vi "Node LUT.vi"(6 "Command":T2, 8 "error in":errorcluster, 9 "node ref":T1, 10 "UID":string) -> (0 "error out":errorcluster, 1 "node ref":T1, 2 "node refs":T1[](array[typedef]), 3 "UIDs":string[](array[string]))   [LabVIEW 2015, in "Node LUT.lvlib"]
uses:
  Node LUT.lvlib
  Command.ctl
  <vilib>/NI/Configuration Framework/Node/NodeRef.ctl
  <vilib>/NI/Configuration Framework/Node/NISE_CEF_Node.lvclass
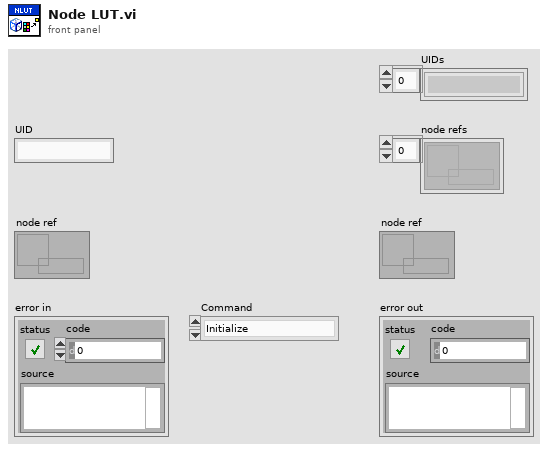
[diagram p1: front panel]
types:
  T1 = typedef "NISE_CEF_Node.lvclass/NodeRef.ctl" = refnum<data-value>
  T2 = typedef "Node LUT.lvlib/Command.ctl" = enum16{"Initialize", "Add Node", "Remove Node", "Node Ref from UID", "List Nodes"}
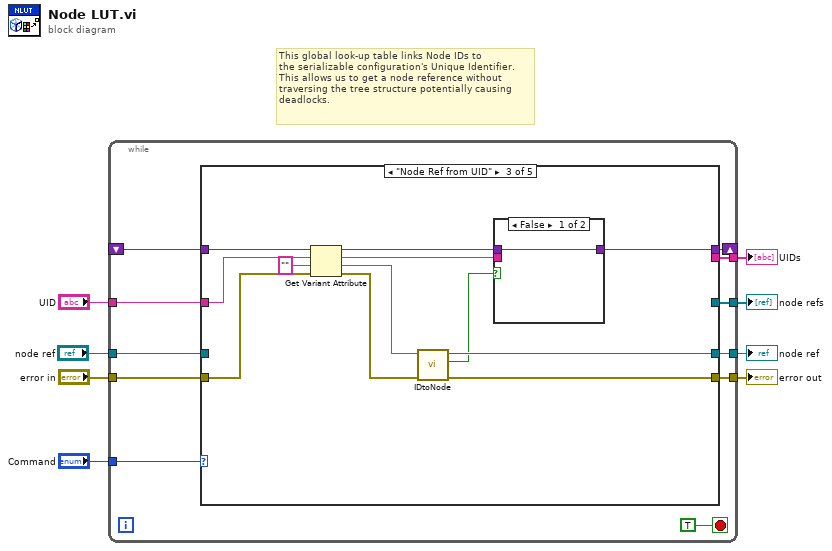
[diagram p0: block diagram]
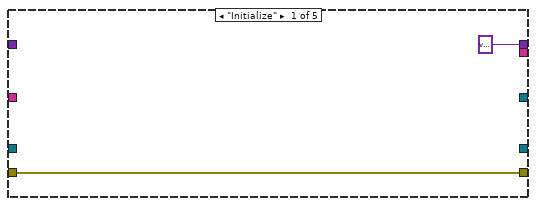
[diagram p2: hidden frame]
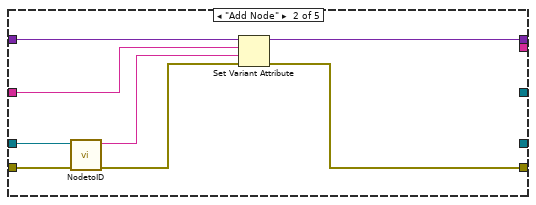
[diagram p3: hidden frame]
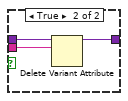
[diagram p4: hidden frame]
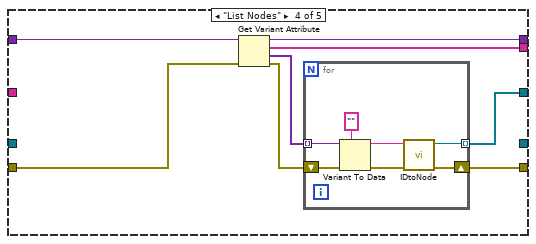
[diagram p5: hidden frame]
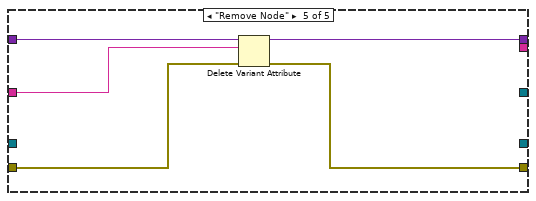
[diagram p6: hidden frame]
diagram:
  # "This global look-up table links Node IDs to\nthe serializable configuration's Unique Identifier.\nThis allows us to get a node reference without\ntraversing the tree structure potentially causing\ndeadlocks."
  n1 = while {
    tunnel: "Command" -> [w18]
    shift-right: [w17] -> _
    shift-left: _ -> [w16]
    tunnel: [w15] -> w7
    tunnel: "error in" -> [w14]
    tunnel: "UID" -> [w13]
    tunnel: "node ref" -> [w12]
    tunnel: [w11] -> w3
    tunnel: [w10] -> w2
    tunnel: [w9] -> w1
    stop <- TRUE stop-if-true
    n2 = case shown="\"Node Ref from UID\"" w18 {
      tunnel: [variant w28 w31 w51 w64] -> w17
      tunnel: w16 -> [_ w29 w40 w52 w60]
      tunnel: [w20 w27 w36 w48 w63] -> w15
      tunnel: w14 -> [w20 w25 w39 w50 w62]
      tunnel: w13 -> [_ w26 w32 _ w61]
      tunnel: w12 -> [_ w22 _ _ _]
      tunnel: [_ _ _ w46 _] -> w11
      tunnel: [_ _ _ w45 _] -> w10
      tunnel: [_ _ w34 _ _] -> w9
      frame "Initialize" {
      }
      frame "Add Node" {
        n3 = call <vilib>:"NodetoID.vi"("error in"=w25, "node ref"=w22) -> ("error out"=w24:errorcluster, "ID"=w23:string)  [unwired: 8 in]
        n4 = Set Variant Attribute(Variant=w29, name=w26, value=w23, error in=w24) -> (Variant out=w28:variant, error out=w27:errorcluster)  [unwired: 1 out]
      }
      frame "Node Ref from UID" {
        n5 = Get Variant Attribute(Variant=w40, name=w32, default value (empty Variant)="", error in=w39) -> (duplicate Variant=w33:variant, value=w35:string, error out=w37:errorcluster)  [unwired: 1 out]
        n6 = call <vilib>:"IDtoNode.vi"("error in"=w37, "ID"=w35) -> ("error out"=w36:errorcluster, "invalid Id"=w30:bool, "node ref"=w34:T1)  [unwired: 7 in]
        n7 = case shown="False" w30 {
          tunnel: w33 -> [w41 w44]
          tunnel: w32 -> [_ w43]
          tunnel: [w41 w42] -> w31
          frame False {
          }
          frame True {
            n8 = Delete Variant Attribute(6:w43, 7:w44) -> (3:w42:variant)  [unwired: 1 in, 2 out]
          }
        }
      }
      frame "List Nodes" {
        n9 = Get Variant Attribute(Variant=w52, error in=w50) -> (duplicate Variant=w51:variant, names=w45:string[], values=w49:variant[], error out=w47:errorcluster)  [unwired: 2 in]
        n10 = for {
          tunnel: w49 -> [w59] mode=indexing
          shift-right: [w54] -> w48
          shift-left: w47 -> [w58]
          tunnel: [w53] -> w46 mode=indexing
          n11 = Variant To Data(error in=w58, type="", Variant=w59) -> (data=w56:string, error out=w55:errorcluster)
          n12 = call <vilib>:"IDtoNode.vi"("error in"=w55, "ID"=w56) -> ("error out"=w54:errorcluster, "node ref"=w53:T1)  [unwired: 7 in, 1 out]
        }
      }
      frame "Remove Node" {
        n13 = Delete Variant Attribute(4:w62, 6:w61, 7:w60) -> (0:w63:errorcluster, 3:w64:variant)  [unwired: 1 out]
      }
    }
  }
  "error out" <- w7
  "node refs" <- w3
  "UIDs" <- w2
  "node ref" <- w1
